vi "AutoHelperSequencer_Example.vi"() -> ()   [LabVIEW 2019]
uses:
  <vilib>/Rock Robotics/WPI/ThirdParty/JAS_Junk/TrajLib/TypeDef/CHASSIS_SPEEDS.ctl
  <vilib>/Rock Robotics/WPI/ThirdParty/JAS_Junk/TrajLib/Enum/AutoHelperSequence_Step_Enum.ctl
  <vilib>/Rock Robotics/WPI/ThirdParty/JAS_Junk/TrajLib/VI/Util_GetTime_U32.vi
  <vilib>/Rock Robotics/WPI/ThirdParty/JAS_Junk/TrajLib/Timer_New.vi
  <vilib>/Rock Robotics/WPI/ThirdParty/JAS_Junk/TrajLib/VI/Util_GetTime_U64.vi
  <vilib>/Utility/semaphor.llb/Obtain Semaphore Reference.vi
  <vilib>/Rock Robotics/WPI/ThirdParty/JAS_Junk/TrajLib/Timer_Reset.vi
  <vilib>/Rock Robotics/WPI/ThirdParty/JAS_Junk/TrajLib/VI/Timer_Restart.vi
  <vilib>/Rock Robotics/WPI/ThirdParty/JAS_Junk/TrajLib/Timer_HasPeriodPassedOnce.vi
  <vilib>/Rock Robotics/WPI/ThirdParty/JAS_Junk/TrajLib/Trajectory_Library.lvlib
panel:
  out "Auto\nRunning":bool
  out "Auto \nFinished":bool
  out "Elapsed Step Time":dbl
  out "Step Number State":T1
  out "Output 2":bool
  out "Output 1":bool
  out "CHASSIS\nSpeed\nDemand":T2 {"vOmega" format="%10.3f"; "vY" format="%10.3f"; "vX" format="%10.3f"}
  in  "Run Auto":bool
  out "Waveform Chart":cluster{i32, i16, i16}(graph)
  # "AUTO HELPER SEQUENCER EXAMPLE"
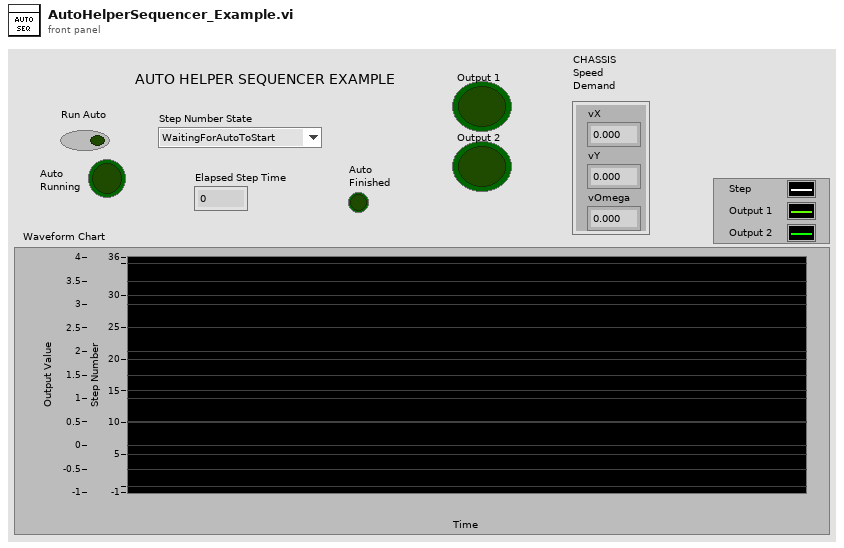
[diagram p1: front panel]
types:
  T1 = typedef "Trajectory_Library.lvlib/AutoHelperSequence_Step_Enum.ctl" = enum16{"WaitingForAutoToStart", "Step 1", "Step 2", "Step 3", "Step 4", "Step 5", "Step 6", "Step 7", "Step 8", "Step 9", "Step 10", "Step 11", "Step 12", "Step 13", "Step 14", "Step 15", "Step 16", "Step 17", "Step 18", "Step 19", "Step 20", "Step 21", "Step 22", "Step 23", "Step 24", "Step 25", "Step 26", "Step 27", "Step 28", "Step 29", "Step 30", "Step 31", "Step 32", "AutoDone"}
  T2 = typedef "Trajectory_Library.lvlib/CHASSIS_SPEEDS.ctl" = cluster{"vX":dbl, "vY":dbl, "vOmega":dbl}
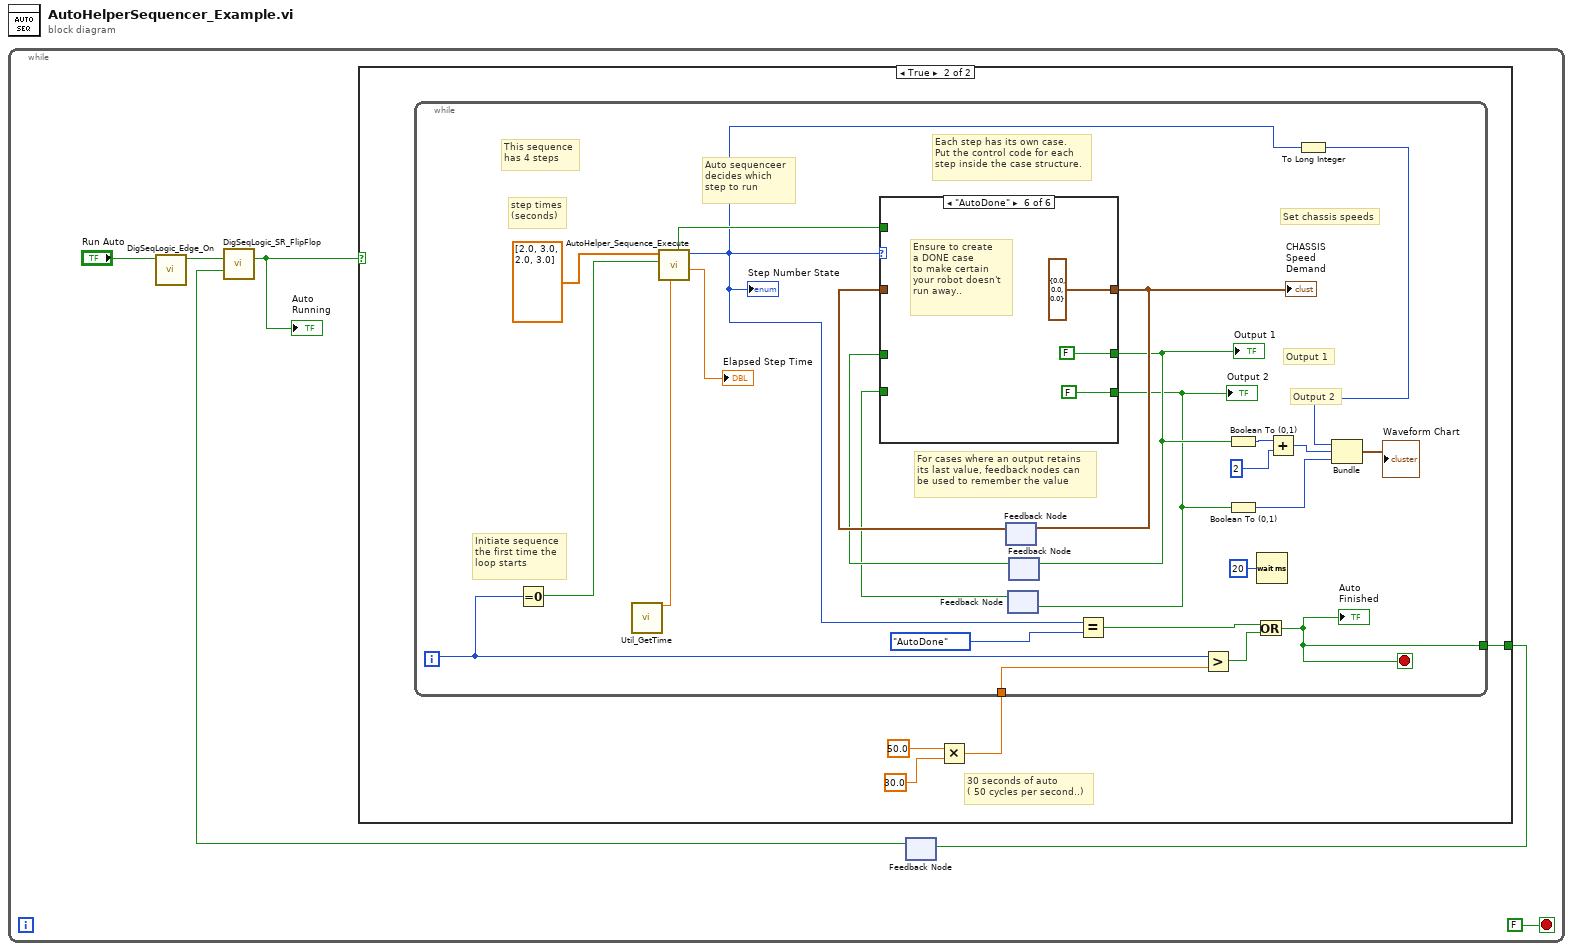
[diagram p0: block diagram]
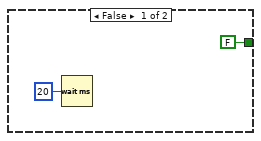
[diagram p2: hidden frame]
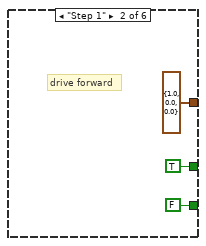
[diagram p4: hidden frame]
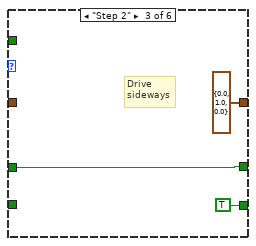
[diagram p5: hidden frame]
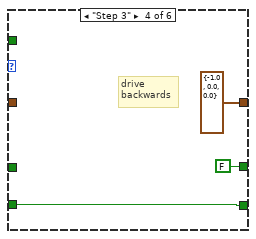
[diagram p6: hidden frame]
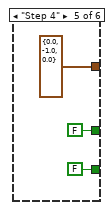
[diagram p7: hidden frame]
diagram:
  n1 = while {
    stop <- FALSE stop-if-true
    n2 = call <vilib>:"DigSeqLogic_Edge_On.vi"("Input"="Run Auto") -> ("On Edge"=w4:bool)  [unwired: 10 in]
    n3 = feedback #1() -> (w1:bool)  [unwired: 1 in]
    n4 = call <vilib>:"DigSeqLogic_SR_FlipFlop.vi"("Set"=w4, "Reset"=w1) -> ("Output"=w3:bool)  [unwired: 12 in, 1 out]
    "Auto\nRunning" <- w3
    n5 = case shown="True" w3 {
      tunnel: [FALSE w9] -> w2
      frame False {
        n6 = Wait (ms)(milliseconds to wait=u32 20) -> ()  [unwired: 1 out]
      }
      frame True {
        # "30 seconds of auto\n( 50 cycles per second..)"
        n7 = Multiply(x=50.0, y=30.0) -> (x*y=w10:dbl)
        n8 = while {
          tunnel: w10 -> [w19]
          tunnel: [w18] -> w9
          i -> [w20]
          stop <- w18 stop-if-true
          # "step times\n(seconds)"
          # "This sequence\nhas 4 steps"
          # "Set chassis speeds"
          # "For cases where an output retains\nits last value, feedback nodes can \nbe used to remember the value"
          # "Output 2"
          # "Output 1"
          # "Each step has its own case.\nPut the control code for each\nstep inside the case structure."
          # "Auto sequenceer\ndecides which\nstep to run"
          # "Initiate sequence\nthe first time the \nloop starts"
          n9 = Equal To 0?(x=w20) -> (x = 0?=w30:bool)
          n10 = call <vilib>:"Util_GetTime.vi"() -> ("FPGA_Time_Seconds"=w29:dbl)  [unwired: 9 in, 2 out]
          n11 = call <vilib>:"AutoHelper_Sequence_Execute.vi"("Pass_Through_Time"=w29, "Initiate"=w30, "Step Times Sec"=dbl[] [2.0, 3.0, 2.0, 3.0]) -> ("Elapsed Step Time"=→"Elapsed Step Time":dbl, "Step Number State"=w14:T1, "New Step"=w22:bool)  [unwired: 4 in, 2 out]
          "Step Number State" <- w14
          n12 = feedback #2() -> (w27:T2)  [unwired: 1 in]
          n13 = feedback #3() -> (w25:bool)  [unwired: 1 in]
          n14 = feedback #4() -> (w26:bool)  [unwired: 1 in]
          n15 = case shown="\"AutoDone\"" w14 {
            tunnel: [w39 TRUE w46 FALSE FALSE FALSE] -> w24
            tunnel: [w40 T2 {"vX"=1.0, "vY"=0.0, "vOmega"=0.0} T2 {"vX"=0.0, "vY"=1.0, "vOmega"=0.0} T2 {"vX"=-1.0, "vY"=0.0, "vOmega"=0.0} T2 {"vX"=0.0, "vY"=-1.0, "vOmega"=0.0} T2 {"vX"=0.0, "vY"=0.0, "vOmega"=0.0}] -> w28
            tunnel: [w38 FALSE TRUE w48 FALSE FALSE] -> w23
            tunnel: w27 -> [w40 _ _ _ _ _]
            tunnel: w26 -> [w39 _ w46 _ _ _]
            tunnel: w25 -> [w38 _ _ w48 _ _]
            tunnel: w22 -> [_ _ _ _ _ _]
            frame "WaitingForAutoToStart", Default {
            }
            frame "Step 1" {
              # "drive forward"
            }
            frame "Step 2" {
              # "Drive \nsideways"
            }
            frame "Step 3" {
              # "drive\nbackwards"
            }
            frame "Step 4" {
            }
            frame "AutoDone" {
              # "Ensure to create\na DONE case\nto make certain\nyour robot doesn't\nrun away.."
            }
          }
          "CHASSIS\nSpeed\nDemand" <- w28
          "Output 1" <- w24
          "Output 2" <- w23
          n16 = feedback-in #2(w28) -> ()
          n17 = feedback-in #3(w23) -> ()
          n18 = feedback-in #4(w24) -> ()
          n19 = Equal?(x=w14, y=AutoHelperSequence_Step_Enum."AutoDone" ("Step Number State")) -> (x = y?=w15:bool)
          n20 = Greater?(x=w20, y=w19) -> (0:w17:bool)
          n21 = Boolean To (0,1)(Boolean=w24) -> (0, 1=w34:i16)
          n22 = Boolean To (0,1)(Boolean=w23) -> (0, 1=w32:i16)
          n23 = Or(x=w15, y=w17) -> (x .or. y?=w18:bool)
          "Auto \nFinished" <- w18
          n24 = Wait (ms)(milliseconds to wait=u32 20) -> ()  [unwired: 1 out]
          n25 = Add(x=w34, y=i16 2) -> (x+y=w33:i16)
          n26 = To Long Integer(number=w14) -> (32bit integer=w13:i32)
          n27 = Bundle(w13, w33, w32) -> (→"Waveform Chart":cluster{i32, i16, i16})  [unwired: 1 in]
        }
      }
    }
    n28 = feedback-in #1(w2) -> ()
  }
